vi "User Event Driver.vi"(11 "error in":errorcluster, 13 "user event operation":T1) -> (4 "stop event reference":refnum<user-event>, 15 "error out":errorcluster)   [LabVIEW 2021, in "Game of Life.lvlib" / "User Event Driver.lvlib"]
uses:
  User Event Driver.lvlib
  User Event Operations.ctl
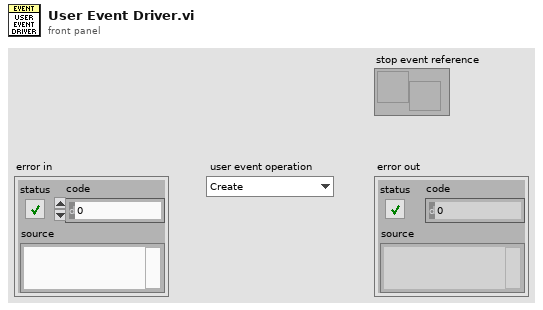
[diagram p1: front panel]
types:
  T1 = typedef "Game of Life.lvlib/User Event Driver.lvlib/User Event Operations.ctl" = enum16{"Create", "Destroy", "Get Reference", "Generate"}
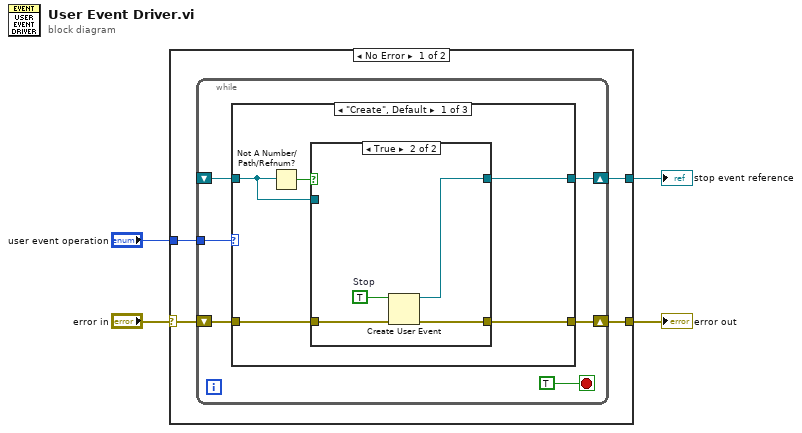
[diagram p0: block diagram]
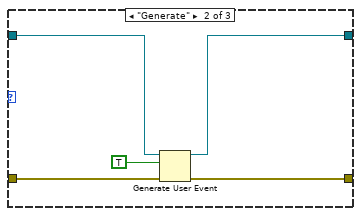
[diagram p3: hidden frame]
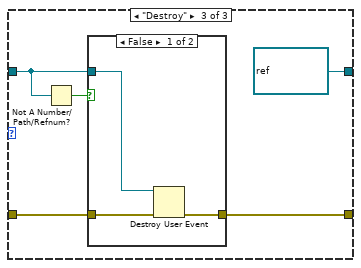
[diagram p4: hidden frame]
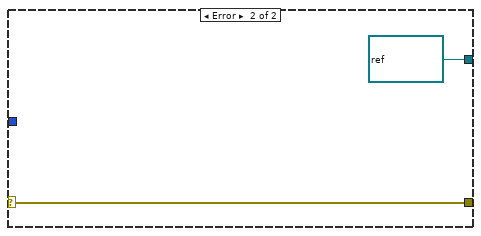
[diagram p6: hidden frame]
diagram:
  n1 = case shown="No Error" "error in" {
    selector: "error in" -> [w5 w41]
    tunnel: [w6 w41] -> w1
    tunnel: "user event operation" -> [w8 _]
    tunnel: [w7 refnum<user-event> refnum ("Stop")] -> w2
    frame No Error {
      n2 = while {
        tunnel: w8 -> [w13]
        shift-right: [w12] -> w7
        shift-left: _ -> [w11]
        shift-right: [w10] -> w6
        shift-left: w5 -> [w9]
        stop <- TRUE stop-if-true
        n3 = case shown="\"Create\", Default" w13 {
          tunnel: [w15 w30 w35] -> w10
          tunnel: w11 -> [w18 w29 w33]
          tunnel: [w17 w27 refnum<user-event> refnum ("Stop")] -> w12
          tunnel: w9 -> [w16 w26 w31]
          frame "Create", Default {
            n4 = Not A Number/Path/Refnum?(number/path/refnum=w18) -> (NaN/Path/Refnum?=w19:bool)
            n5 = case shown="True" w19 {
              tunnel: w16 -> [w21 w23]
              tunnel: [w21 w22] -> w15
              tunnel: w18 -> [w20 _]
              tunnel: [w20 w24] -> w17
              frame False {
              }
              frame True {
                w25 = TRUE  # Stop
                n6 = Create User Event(user event datatype=w25, error in=w23) -> (user event=w24:refnum<user-event>, error out=w22:errorcluster)
              }
            }
          }
          frame "Generate" {
            n7 = Generate User Event(user event=w29, event data cluster=TRUE ("event data"), error in=w26) -> (user event out=w27:refnum<user-event>, error out=w30:errorcluster)  [unwired: 1 in]
          }
          frame "Destroy" {
            n8 = Not A Number/Path/Refnum?(number/path/refnum=w33) -> (NaN/Path/Refnum?=w34:bool)
            n9 = case shown="False" w34 {
              tunnel: w31 -> [w36 w39]
              tunnel: [w37 w39] -> w35
              tunnel: w33 -> [w38 _]
              frame False {
                n10 = Destroy User Event(user event=w38, error in=w36) -> (error out=w37:errorcluster)
              }
              frame True {
              }
            }
          }
        }
      }
    }
    frame Error {
    }
  }
  "error out" <- w1
  "stop event reference" <- w2
